vi "Format Time for RPI.vi"() -> (2 "is date valid?":bool, 3 "date/time string":string)   [LabVIEW 2025]
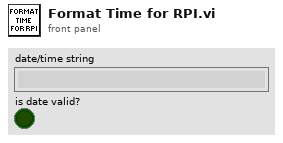
[diagram p1: front panel]
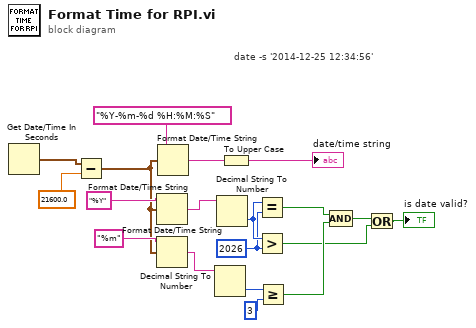
[diagram p0: block diagram]
diagram:
  w14 = 2026 ("y")
  # "date -s '2014-12-25 12:34:56'"
  n1 = Get Date/Time In Seconds() -> (seconds since 1Jan1904=w2:timestamp)
  n2 = Subtract(x=w2, y=21600.0) -> (x-y=w1:timestamp)
  n3 = Format Date/Time String(time format string (%c)="%Y", seconds (now)=w1) -> (date/time string=w16:string)  [unwired: 1 in]
  n4 = Format Date/Time String(time format string (%c)="%m", seconds (now)=w1) -> (date/time string=w13:string)  [unwired: 1 in]
  n5 = Format Date/Time String(time format string (%c)="%Y-%m-%d %H:%M:%S", seconds (now)=w1) -> (date/time string=w5:string)  [unwired: 1 in]
  n6 = Decimal String To Number(string=w13) -> (number=w12:i32)  [unwired: 2 in, 1 out]
  n7 = Decimal String To Number(string=w16) -> (number=w15:i32)  [unwired: 2 in, 1 out]
  n8 = To Upper Case(1:w5) -> (0:→"date/time string":string)
  n9 = Equal?(x=w15, y=w14) -> (x = y?=w10:bool)
  n10 = Greater?(x=w15, y=w14) -> (0:w7:bool)
  n11 = Greater Or Equal?(x=w12, y=3) -> (x >= y?=w9:bool)
  n12 = Compound Arithmetic op=AND(w10, w9) -> (w8:bool)
  n13 = Or(x=w8, y=w7) -> (x .or. y?=→"is date valid?":bool)
